vi "RemoveChannel.vi"(8 "error in (no error)":errorcluster, 10 "Name":string, 11 "object in":refnum<class "ChannelManagerUI.lvclass">) -> (0 "error out":errorcluster, 3 "object out":refnum<class "ChannelManagerUI.lvclass">)   [LabVIEW 2021, in "Channel.lvlib" / "ChannelManagerUI.lvlib" / "ChannelManagerUI.lvclass"]
doc: "Adds the channel"
uses:
  ChannelManagerUI.lvclass
  ChannelsManager/ChannelsManager/ChannelsManager.lvclass
  ChannelManagerUI.lvclass/ChannelManagerUI.ctl
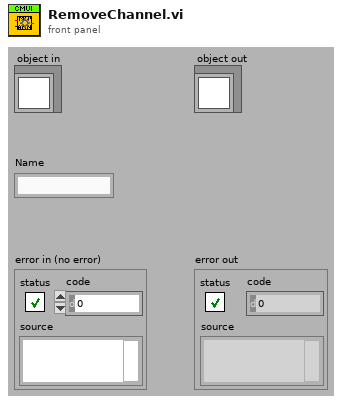
[diagram p1: front panel]
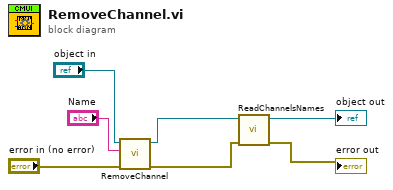
[diagram p0: block diagram]
diagram:
  n1 = call-parent "RemoveChannel.vi"("error in (no error)"="error in (no error)", "Name"="Name", "object in"="object in") -> ("error out"=w2:errorcluster, "object out"=w7:refnum<class "ChannelManagerUI.lvclass">)  [unwired: 7 in]
  n2 = call-dynamic "ReadChannelsNames.vi"("error in (no error)"=w2, "ChannelManagerUI in"=w7) -> ("error out"=→"error out":errorcluster, "ChannelManagerUI out"=→"object out":refnum<class "ChannelManagerUI.lvclass">)  [unwired: 7 in, 1 out]
